vi "Create (New).vi"(6 "Config Version (0.0.0)":string="0.0.0", 8 "error in (no error)":errorcluster) -> (0 "error out":errorcluster, 3 "VolatusConfig out":refnum<class "VolatusConfig.lvclass">)   [LabVIEW 2020, in "VolatusConfig.lvlib" / "VolatusConfig.lvclass"]
uses:
  VolatusConfig.lvclass
  lv-cdm/CDM-Config/Config Manager/Config Manager.lvclass/Config Manager.ctl
  VolatusConfig.lvclass/VolatusConfig.ctl
  lv-cdm/CDM-Config/Config Element/Set Owner.vi
  lv-cdm/CDM-Config/Config Element/Config Element.lvclass
  lv-cdm/CDM-Config/Config Manager/Config Manager.lvclass
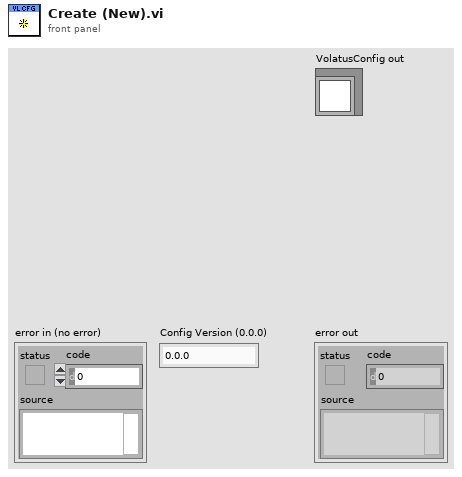
[diagram p1: front panel]
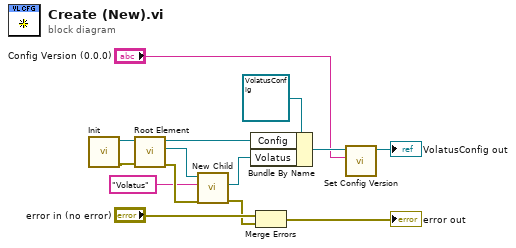
[diagram p0: block diagram]
diagram:
  n1 = call "Init.vi"() -> ("error out"=w7:errorcluster, "Config Manager out"=w11:refnum<class "Config Manager.lvclass">)  [unwired: 10 in]
  n2 = call "Root Element.vi"("error in (no error)"=w7, "Config Manager in"=w11) -> ("error out"=w14:errorcluster, "Root Element"=w9:refnum<class "Config Element.lvclass">, "Config Manager out"=w10:refnum<class "Config Manager.lvclass">)  [unwired: 7 in]
  n3 = call "New Child.vi"("error in (no error)"=w14, "Child Name"="Volatus", "Config Element in"=w9) -> ("error out"=w2:errorcluster, "New Child"=w1:refnum<class "Config Element.lvclass">)  [unwired: 6 in, 1 out]
  n4 = Bundle By Name(cluster=refnum<class "VolatusConfig.lvclass"> refnum ("VolatusConfig in"), "Config"=w10, "Volatus"=w1) -> (w5:refnum<class "VolatusConfig.lvclass">)
  n5 = Merge Errors("error in (no error)", w2) -> (→"error out":errorcluster)
  n6 = call "Set Config Version.vi"("Config Version"="Config Version (0.0.0)", "VolatusConfig in"=w5) -> ("VolatusConfig out"=→"VolatusConfig out":refnum<class "VolatusConfig.lvclass">)  [unwired: 8 in, 1 out]
